vi "GetConfigurationType.vi"(8 "error in (no error)":errorcluster, 11 "object in":refnum<class "Type_Channel.lvclass">) -> (0 "error out":errorcluster, 2 "Configuration":refnum<class "Configuration.lvclass">, 3 "object out":refnum<class "Type_Channel.lvclass">)   [LabVIEW 2021, in "Template-Channels.lvlib" / "Type_Channel.lvclass"]
doc: "Gets the Configuration to use"
uses:
  Type_Channel.lvclass
  Dependencies/Channel.lvlibp/Channel/Configuration_class/Configuration.lvclass
  Template_CFG/Template_CFG.lvclass
  C:/Users/averna/Documents/LV Gym DEMO/Factory Pattern/Channels/Dependencies/Channel.lvlibp/Channel/Configuration_class/Configuration.lvclass
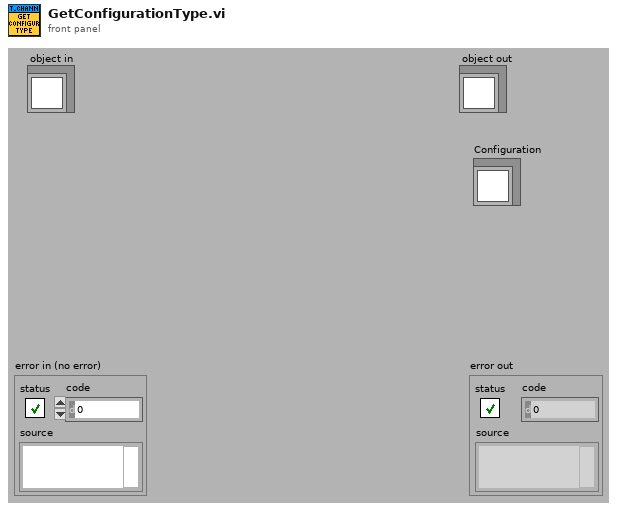
[diagram p1: front panel]
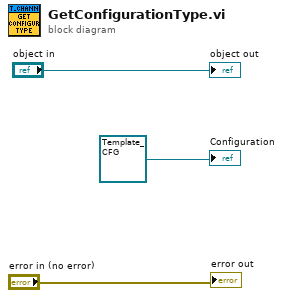
[diagram p0: block diagram]
diagram:
  "error out" <- "error in (no error)"
  "object out" <- "object in"
  "Configuration" <- refnum<class "Template_CFG.lvclass"> refnum ("Template-Channels.lvlib:Template_CFG")
